vi "test.vi"   [LabVIEW 2016, in "13.03 Robot.lvrbt"]
uses:
  13.03 Robot.lvrbt
  <vilib>/NXT/Block Support/NXT_OutputPort.ctl
  <vilib>/NXT/NXTIO Xnodes/NXTIONodeSubVIs/NXTMoveMotors.vi
  <vilib>/NXT/Subs/LVHSConnector.ctl
  <vilib>/NXT/NXTIO Xnodes/AddressXNode/NXTIOAddress.xnode
  <vilib>/NXT/NXTIO Xnodes/NXTIOXNode/NXTIO.xnode
  <vilib>/NXT/LegoClasses/BrickReference/BrickReference.lvclass
types:
  T1 = typedef "NXT_OutputPort.ctl" = u8
  T2 = typedef "LVHSConnector.ctl" = refnum<class "BrickReference.lvclass">
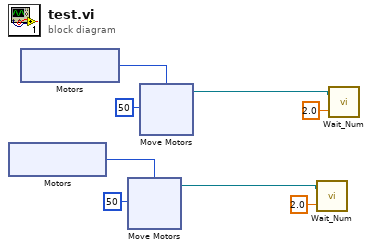
[diagram p0: block diagram]
diagram:
  n1 = xnode "Motors"() -> ("Motor"=w2:T1)
  n2 = xnode "Motors"() -> ("Motor"=w6:T1)
  n3 = xnode "Move Motors"("Power/Speed 1"=i8 50, "Motors"=w2) -> ("NXT/EV3"=w4:T2)  [unwired: 1 in]
  n4 = xnode "Move Motors"("Power/Speed 1"=i8 50, "Motors"=w6) -> ("NXT/EV3"=w8:T2)  [unwired: 1 in]
  n5 = call <vilib>:"Wait_Num.vi"("Time (1 sec)"=sgl 2.0, "NXT/EV3"=w4) -> ()  [unwired: 2 in, 1 out]
  n6 = call <vilib>:"Wait_Num.vi"("Time (1 sec)"=sgl 2.0, "NXT/EV3"=w8) -> ()  [unwired: 2 in, 1 out]
